vi "Compute Time Remaining.vi"(8 "error in (no error)":errorcluster, 11 "Dialog in":refnum<class "Dialog.lvclass">) -> (0 "error out":errorcluster, 1 "Elapsed":bool, 2 "Time remaining (s)":dbl, 3 "Dialog out":refnum<class "Dialog.lvclass">)   [LabVIEW 2012, in "Dialog.lvlib" / "Dialog.lvclass"]
uses:
  Dialog.lvclass
  Dialog.lvclass/Dialog.ctl
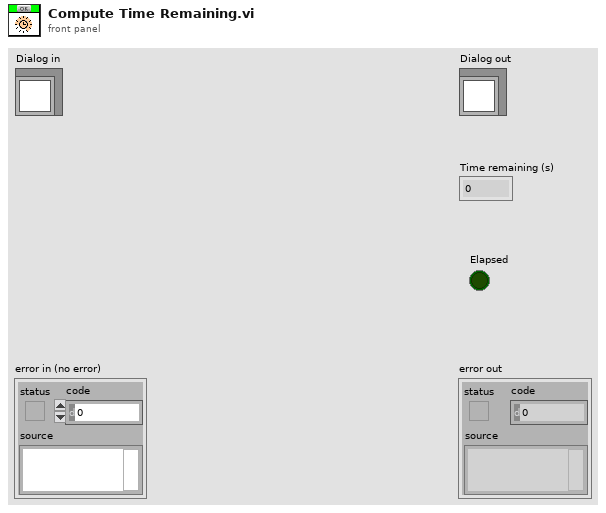
[diagram p1: front panel]
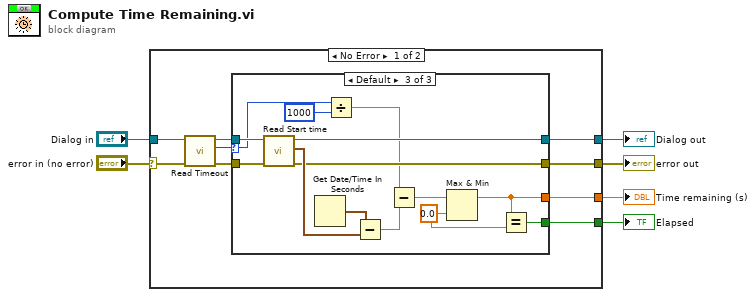
[diagram p0: block diagram]
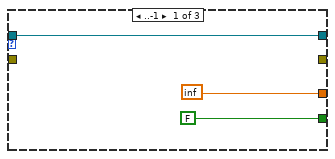
[diagram p2: hidden frame]
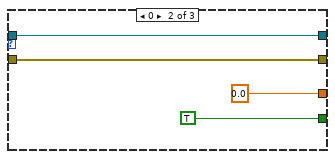
[diagram p3: hidden frame]
diagram:
  n1 = case shown="No Error" "error in (no error)" {
    selector: "error in (no error)" -> [w8 w38]
    tunnel: [w7 w38] -> w5
    tunnel: [w13 w37] -> w3
    tunnel: "Dialog in" -> [w15 w37]
    tunnel: [w11 _] -> w2
    tunnel: [w10 _] -> w1
    frame No Error {
      n2 = call-dynamic "Read Timeout.vi"("error in (no error)"=w8, "Dialog.lvclass in"=w15) -> ("error out"=w9:errorcluster, "Timeout"=w12:i32, "Dialog.lvclass out"=w14:refnum<class "Dialog.lvclass">)  [unwired: 7 in]
      n3 = case shown="Default" w12 {
        selector: w12 -> [_ _ w31]
        tunnel: w14 -> [w18 w22 w36]
        tunnel: [w18 w22 w35] -> w13
        tunnel: [FALSE TRUE w25] -> w11
        tunnel: [inf 0.0 w23] -> w10
        tunnel: w9 -> [_ w20 w33]
        tunnel: [_ w20 w32] -> w7
        frame ..-1 {
        }
        frame 0 {
        }
        frame Default {
          w24 = 0.0 ("y")
          n4 = call "Read Start time.vi"("error in (no error)"=w33, "Dialog in"=w36) -> ("error out"=w32:errorcluster, "Start time"=w34:timestamp, "Dialog out"=w35:refnum<class "Dialog.lvclass">)  [unwired: 7 in]
          n5 = Get Date/Time In Seconds() -> (seconds since 1Jan1904=w29:timestamp)
          n6 = Divide(x=w31, y=1000) -> (x/y=w28:dbl)
          n7 = Subtract(x=w29, y=w34) -> (x-y=w27:dbl)
          n8 = Subtract(x=w28, y=w27) -> (x-y=w26:dbl)
          n9 = Max & Min(x=w26, y=w24) -> (max(x,y)=w23:dbl)  [unwired: 1 out]
          n10 = Equal?(x=w23, y=w24) -> (x = y?=w25:bool)
        }
      }
    }
    frame Error {
    }
  }
  "error out" <- w5
  "Dialog out" <- w3
  "Time remaining (s)" <- w1
  "Elapsed" <- w2
